vi "Publish Values.vi"(8 "error in (no error)":errorcluster, 11 "SoftVar Module in":refnum<class "SoftVar Module.lvclass">) -> (0 "error out":errorcluster, 3 "SoftVar Module out":refnum<class "SoftVar Module.lvclass">)   [LabVIEW 2020, in "Volatus.lvlib" / "SoftVar Module.lvclass"]
uses:
  SoftVar Module.lvclass
  C:/dev/lv20CE/relink/lv-volatus/Volatus/Module/Module.lvclass
  SoftVar Module.lvclass/SoftVar Module.ctl
  Module/Module.lvclass/Module.ctl
  VolatusAPI/VolatusAPI.lvclass/VolatusAPI.ctl
  lv-vecto/Vecto/Group DBL/Group DBL.lvclass
  C:/dev/lv20CE/relink/lv-vecto/Vecto/Group/Group.lvclass
  Module/Module.lvclass
  VolatusAPI/VolatusAPI.lvclass
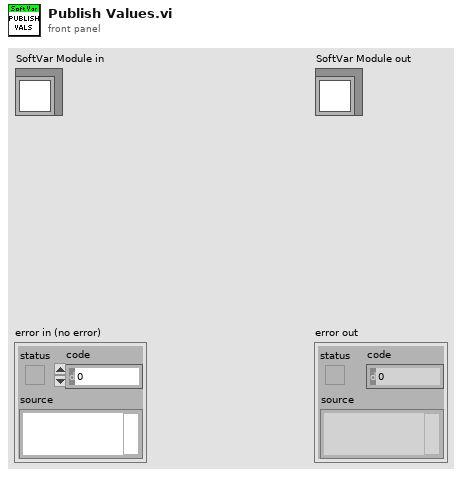
[diagram p1: front panel]
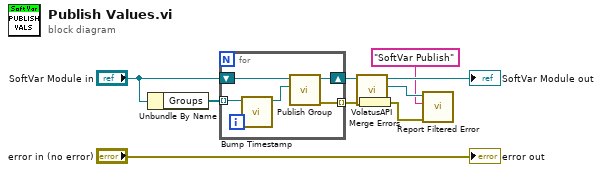
[diagram p0: block diagram]
diagram:
  n1 = Unbundle By Name("SoftVar Module in") -> ("Groups"=w6:refnum<class "Group DBL.lvclass">[])
  n2 = for {
    shift-right: [w13] -> w7
    shift-left: "SoftVar Module in" -> [w14]
    tunnel: w6 -> [w10] mode=indexing
    tunnel: [w12] -> w4 mode=indexing
    n3 = call "Bump Timestamp.vi"("Group in"=w10) -> ("Group out"=w11:refnum<class "Group DBL.lvclass">)  [unwired: 9 in, 1 out]
    n4 = call "Publish Group.vi"("Group"=w11, "Module in"=w14) -> ("error out"=w12:errorcluster, "Module out"=w13:refnum<class "SoftVar Module.lvclass">)  [unwired: 8 in]
  }
  n5 = call "VolatusAPI.vi"("Module in"=w7) -> ("VolatusAPI"=w2:refnum<class "VolatusAPI.lvclass">, "Module out"=→"SoftVar Module out":refnum<class "SoftVar Module.lvclass">)  [unwired: 9 in]
  n6 = Merge Errors(w4) -> (w3:errorcluster)
  n7 = call "Report Filtered Error.vi"("error in (no error)"=w3, "Context"="SoftVar Publish", "VolatusAPI in"=w2) -> ()  [unwired: 7 in, 2 out]
  "error out" <- "error in (no error)"
